vi "set Reference Level Offset.vi"(8 "error in (no error)":errorcluster, 10 "Reference Level Offset":dbl, 11 "FSV-40N in":refnum<class "FSV-40N.lvclass">) -> (0 "error out":errorcluster, 3 "FSV-40N out":refnum<class "FSV-40N.lvclass">)   [LabVIEW 2023, in "Spectrum Analyzer.lvlib" / "FSV-40N.lvclass"]
uses:
  FSV-40N.lvclass
  FSV-40N.lvclass/FSV-40N.ctl
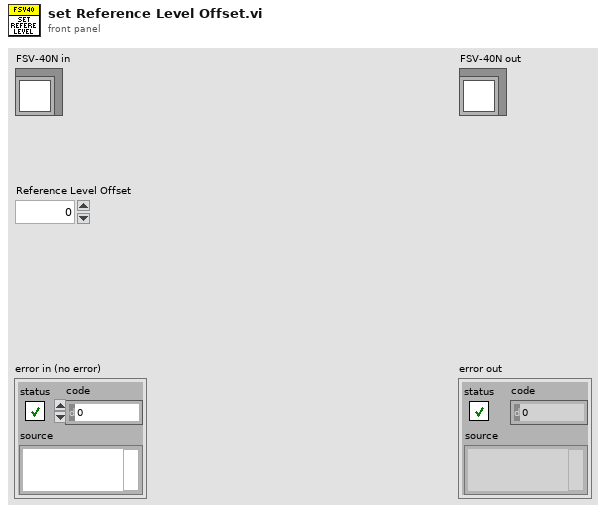
[diagram p1: front panel]
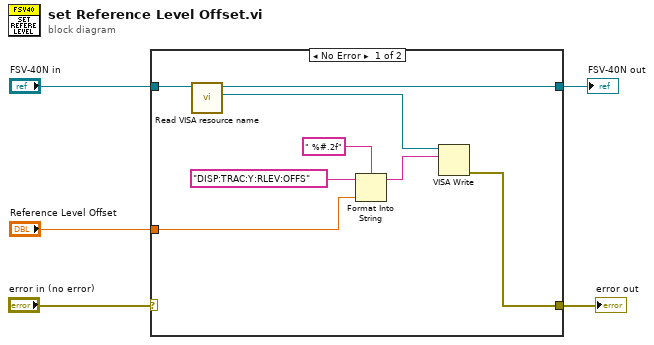
[diagram p0: block diagram]
diagram:
  n1 = case shown="No Error" "error in (no error)" {
    selector: "error in (no error)" -> [_ w14]
    tunnel: "FSV-40N in" -> [w13 w15]
    tunnel: [w11 w15] -> w4
    tunnel: [w10 w14] -> w2
    tunnel: "Reference Level Offset" -> [w7 _]
    frame No Error {
      n2 = call "Read VISA resource name.vi"("FSV-40N in"=w13) -> ("VISA resource name"=w12:refnum<visa-resource-name>, "FSV-40N out"=w11:refnum<class "FSV-40N.lvclass">)  [unwired: 8 in, 1 out]
      n3 = Format Into String(format string=" %#.2f", initial string="DISP:TRAC:Y:RLEV:OFFS" ("write buffer"), w7) -> (resulting string=w6:string)  [unwired: 1 in, 1 out]
      n4 = VISA Write(VISA resource name=w12, write buffer=w6) -> (error out=w10:errorcluster)  [unwired: 1 in, 2 out]
    }
    frame Error {
    }
  }
  "error out" <- w2
  "FSV-40N out" <- w4
